vi "Read Numeric Limits.vi"(9 "schema type":string, 10 "default value":variant, 11 "control":refnum<vi>) -> (1 "unit note":string, 2 "maximum":string, 3 "minimum":string)   [LabVIEW 2020, in "MCP Server.lvlib"]
doc: "Reads the minimum, maximum and unit of a numeric control for its JSON Schema, for Add Control Details To Schema.vi. An integer gets the range of its representation (written as exact integers), a number none: the data entry limits replace these where they are tighter and not set to Ignore. A number with a unit gets \"Unit: <unit>.\" as unit note. Bounds and unit note are JSON text, empty where there is none. Any other schema type gets nothing."
uses:
  MCP Server.lvlib
  c4f94649-146f-4d8a-90e2-51f4313f99c1.vi
  c3b01861-0ed8-4dd5-b426-f21d792e956a.vi
  <vilib>/JDP Science/JSONtext/Variant to JSON Text.vi
  <vilib>/JDP Science/JSONtext/LVClass Serializer/JSONtext LVClass Serializer.lvclass
  <vilib>/Utility/Data Type/NI_Data Type.lvlib
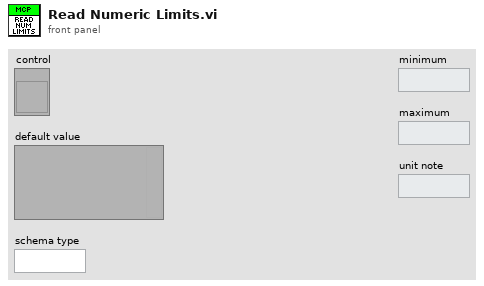
[diagram p1: front panel]
types:
  T1 = typedef "LVNumericRepresentation.ctl" = enum32{"Extended Precision", "Double Precision", "Single Precision", "Long", "Word", "Byte", "Unsigned Long", "Unsigned Word", "Unsigned Byte", "Complex Extended", "Complex Double", "Complex Single", "Quad", "Unsigned Quad", "Fixed-Point"}
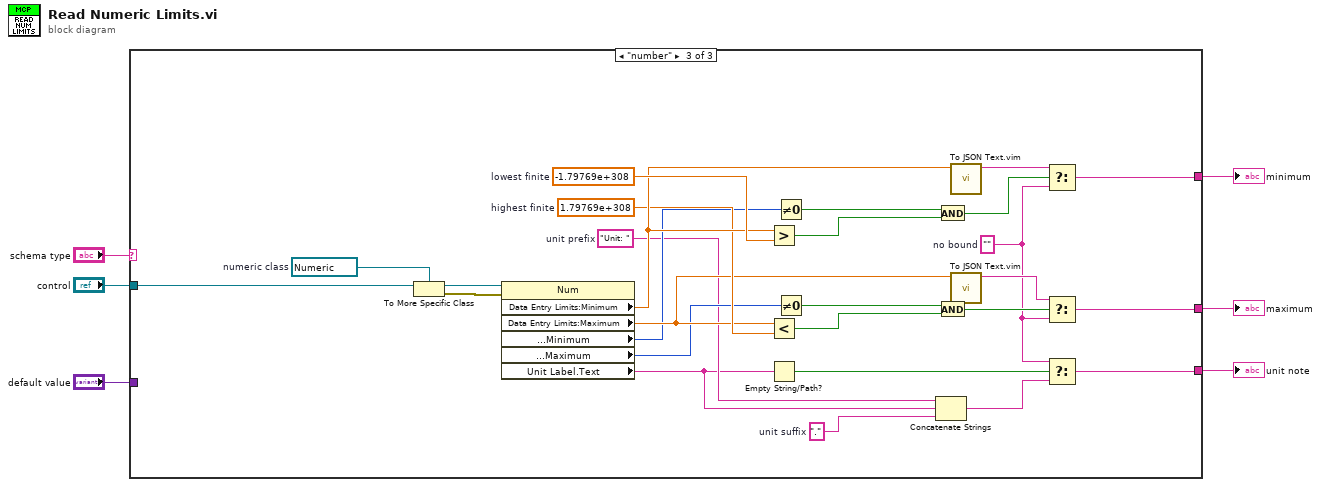
[diagram p0: block diagram]
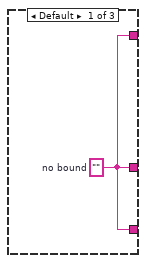
[diagram p2: hidden frame]
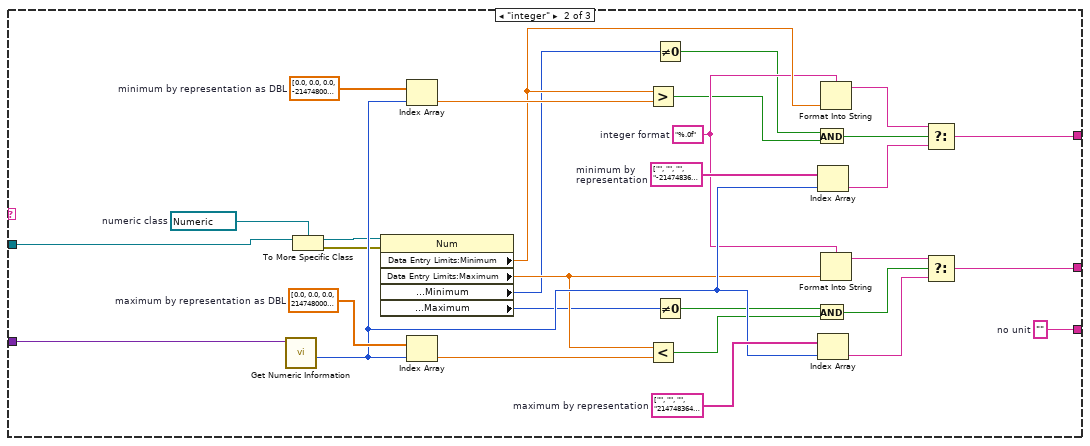
[diagram p3: hidden frame]
diagram:
  n1 = case shown="\"number\"" "schema type" {
    tunnel: "control" -> [_ w36 w64]
    tunnel: "default value" -> [_ w37 _]
    tunnel: [w7 w10 w40] -> w3
    tunnel: [w7 w9 w39] -> w2
    tunnel: [w7 w8 w38] -> w1
    frame Default {
      w7 = ""  # no bound
    }
    frame "integer" {
      w8 = ""  # no unit
      w23 = "%.0f"  # integer format
      w31 = dbl[] [0.0, 0.0, 0.0, 2147480000.0, 32767.0, 127.0, 4294970000.0, 65535.0, 255.0, 0.0, 0.0, 0.0, 9.22337e+18, 1.84467e+19, 0.0]  # maximum by representation as DBL
      w32 = dbl[] [0.0, 0.0, 0.0, -2147480000.0, -32768.0, -128.0, 0.0, 0.0, 0.0, 0.0, 0.0, 0.0, -9.22337e+18, 0.0, 0.0]  # minimum by representation as DBL
      w33 = string[] ["", "", "", "2147483647", "32767", "127", "4294967295", "65535", "255", "", "", "", "9223372036854775807", "18446744073709551615", ""]  # maximum by representation
      w34 = string[] ["", "", "", "-2147483648", "-32768", "-128", "0", "0", "0", "", "", "", "-9223372036854775808", "0", ""]  # minimum by representation
      w35 = refnum<vi> refnum  # numeric class
      n2 = call <vilib>:"Get Numeric Information.vi"("variant"=w37) -> ("representation"=w30:T1)  [unwired: 7 in, 3 out]
      n3 = To More Specific Class(target class=w35, reference=w36) -> (specific class reference=w29:refnum<vi>, error out=w28:errorcluster)  [unwired: 1 in]
      n4 = property class="Num"(reference=w29, error in=w28) -> ("Data Entry Limits:Minimum"=w26:dbl, "Data Entry Limits:Maximum"=w24:dbl, "Response to Value Outside Limits:Minimum"=w22:u8, "Response to Value Outside Limits:Maximum"=w21:u8)  [unwired: 2 out]
      n5 = Index Array(array=w32, index=w30) -> (element=w27:dbl)
      n6 = Index Array(array=w31, index=w30) -> (element=w25:dbl)
      n7 = Greater?(x=w26, y=w27) -> (0:w19:bool)
      n8 = Less?(x=w24, y=w25) -> (x < y?=w17:bool)
      n9 = Not Equal To 0?(x=w22) -> (x != 0?=w20:bool)
      n10 = Not Equal To 0?(x=w21) -> (x != 0?=w18:bool)
      n11 = And(x=w20, y=w19) -> (x .and. y?=w15:bool)
      n12 = And(x=w18, y=w17) -> (x .and. y?=w12:bool)
      n13 = Index Array(array=w34, index=w30) -> (element=w14:string)
      n14 = Index Array(array=w33, index=w30) -> (element=w11:string)
      n15 = Format Into String(format string=w23, w26) -> (resulting string=w16:string)  [unwired: 2 in, 1 out]
      n16 = Format Into String(format string=w23, w24) -> (resulting string=w13:string)  [unwired: 2 in, 1 out]
      n17 = Select(t=w16, s=w15, f=w14) -> (s? t:f=w10:string)
      n18 = Select(t=w13, s=w12, f=w11) -> (s? t:f=w9:string)
    }
    frame "number" {
      w52 = "."  # unit suffix
      w54 = "Unit: "  # unit prefix
      w41 = ""  # no bound
      w58 = 1.79769e+308  # highest finite
      w60 = -1.79769e+308  # lowest finite
      w63 = refnum<vi> refnum  # numeric class
      n19 = To More Specific Class(target class=w63, reference=w64) -> (specific class reference=w62:refnum<vi>, error out=w61:errorcluster)  [unwired: 1 in]
      n20 = property class="Num"(reference=w62, error in=w61) -> ("Data Entry Limits:Minimum"=w59:dbl, "Data Entry Limits:Maximum"=w57:dbl, "Response to Value Outside Limits:Minimum"=w56:u8, "Response to Value Outside Limits:Maximum"=w55:u8, "Unit Label.Text"=w53:string)  [unwired: 2 out]
      n21 = Greater?(x=w59, y=w60) -> (0:w50:bool)
      n22 = Less?(x=w57, y=w58) -> (x < y?=w48:bool)
      n23 = Empty String/Path?(string/path=w53) -> (empty?=w47:bool)
      n24 = Not Equal To 0?(x=w56) -> (x != 0?=w51:bool)
      n25 = Not Equal To 0?(x=w55) -> (x != 0?=w49:bool)
      n26 = Concatenate Strings(w54, w53, w52) -> (w46:string)
      n27 = And(x=w51, y=w50) -> (x .and. y?=w44:bool)
      n28 = And(x=w49, y=w48) -> (x .and. y?=w42:bool)
      n29 = call "To JSON Text.vim"("Anything"=w59) -> ("<JSON>"=w45:string)  [unwired: 9 in, 1 out]
      n30 = call "To JSON Text.vim"("Anything"=w57) -> ("<JSON>"=w43:string)  [unwired: 9 in, 1 out]
      n31 = Select(t=w45, s=w44, f=w41) -> (s? t:f=w40:string)
      n32 = Select(t=w43, s=w42, f=w41) -> (s? t:f=w39:string)
      n33 = Select(t=w41, s=w47, f=w46) -> (s? t:f=w38:string)
    }
  }
  "minimum" <- w3
  "maximum" <- w2
  "unit note" <- w1
